vi "Process IMAQ Image (Webcam).vi"() -> ()   [LabVIEW 2020]
uses:
  <vilib>/userDefined/High Color/IMAQdx.ctl
  <vilib>/vision/driver/IMAQdx.llb/IMAQdx Buffer Number Mode.ctl
  6d5f1638-640c-4e20-b011-0cee3ae60b95.vi
  688a6956-cd2d-4b8a-a8be-e172edc5432f.vi
  45820c2d-b3f1-45d5-9983-17417cdda85c.vi
  G-Embedded-Python-Interpreter-Toolkit/Null Py Object Refnum.vi
  6d5f1638-640c-4e20-b011-0cee3ae60b95.vi/96ddca92-7bbf-40e2-a1a5-d32f291eb6af.vi
  G-Embedded-Python-Interpreter-Toolkit-IMAQ/IMAQ to Py Object.vi/22f05568-5bba-4402-9e98-aca160827363.vi
  688a6956-cd2d-4b8a-a8be-e172edc5432f.vi/6c7a13f1-33d3-431d-8188-904cac5422b3.vi
  45820c2d-b3f1-45d5-9983-17417cdda85c.vi/6c7a13f1-33d3-431d-8188-904cac5422b3.vi
  G-Embedded-Python-Interpreter-Toolkit/Python Object Reference to Pointer Sized Ref.vi
  G-Embedded-Python-Interpreter-Toolkit/Pointer Sized Ref to Python Object Reference.vi
  G-Embedded-Python-Interpreter-Toolkit/Merge Call Library Errors.vi
  G-Embedded-Python-Interpreter-Toolkit/Generate Argument Type Info.vi
  G-Embedded-Python-Interpreter-Toolkit/Create Py Object IMAQ Image.vi
  G-Embedded-Python-Interpreter-Toolkit/G-Embedded-Python-Interpreter-Toolkit.lvlib
  G-Embedded-Python-Interpreter-Toolkit-IMAQ/G-Embedded-Python-Interpreter-Toolkit-IMAQ.lvlib
  <vilib>/vision/driver/NI_Vision_Acquisition_Software.lvlib
panel:
  in  "stop":bool
  out "Image":T1(plugin-control)
  in  "Session In":T2="cam0"
  out "Print Ouptut":string
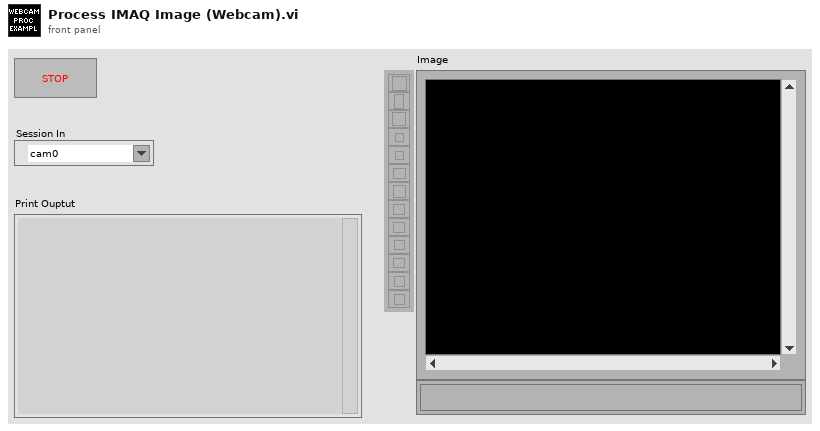
[diagram p1: front panel]
types:
  T1 = typedef "IMAQ Image.ctl" = refnum<image>
  T2 = typedef "IMAQdx.ctl" = refnum<k21>
  T3 = typedef "Image Type" = u32
  T4 = typedef "G-Embedded-Python-Interpreter-Toolkit.lvlib/Python Object Reference.ctl" = refnum<k1>
  T5 = typedef "NI_Vision_Acquisition_Software.lvlib/IMAQdx Buffer Number Mode.ctl" = enum32{"Next", "Last", "Buffer Number", "Every", "Last New"}
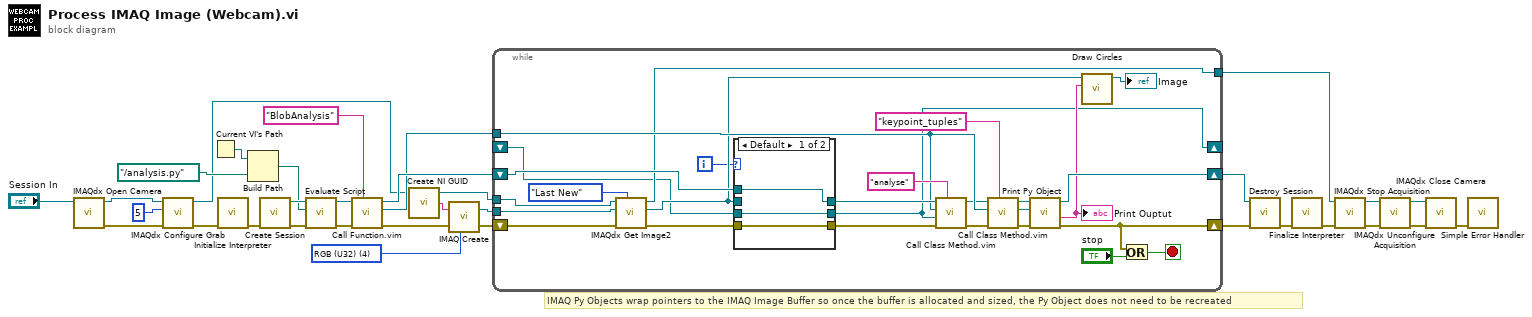
[diagram p0: block diagram]
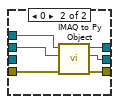
[diagram p2: hidden frame]
diagram:
  w23 = T3 4 items=["Grayscale (U8)", "Grayscale (I16)", "Grayscale (SGL)", "Complex (CSG)", "RGB (U32)", "HSL (U32)", "RGB (U64)", "Grayscale (U16)"] ("Image Type")
  # "IMAQ Py Objects wrap pointers to the IMAQ Image Buffer so once the buffer is allocated and sized, the Py Object does not need to be recreated"
  n1 = call <vilib>:"IMAQdx Open Camera.vi"("Session In"="Session In") -> ("error out"=w11:errorcluster, "Session Out"=w12:T2)  [unwired: 9 in]
  n2 = call <vilib>:"IMAQdx Configure Grab.vi"("error in"=w11, "Number of Buffers"=u32 5, "Session In"=w12) -> ("error out"=w9:errorcluster, "Session Out"=w8:T2)  [unwired: 7 in]
  n3 = Current VI's Path() -> (path=w21:path)
  n4 = call "Initialize Interpreter.vi"("error in (no error)"=w9) -> ("error out"=w32:errorcluster)  [unwired: 9 in, 1 out]
  n5 = Build Path(base path=w21, name or relative path=path "../analysis.py") -> (appended path=w28:path)
  n6 = call "Create Session.vi"("error in (no error)"=w32) -> ("error out"=w31:errorcluster, "Session Handle"=w30:refnum<data-value>)  [unwired: 9 in]
  n7 = call "Evaluate Script.vi"("error in (no error)"=w31, "Script File Path"=w28, "Session Handle in"=w30) -> ("error out"=w25:errorcluster, "Session Handle out"=w26:refnum<data-value>)  [unwired: 7 in]
  n8 = call "Call Function.vim"("Function Name"="BlobAnalysis", "error in (no error)"=w25, "Data Value Reference in"=w26) -> ("error out"=w22:errorcluster, "Returned Python Object Refnum"=w18:T4, "Data Value Reference out"=w20:refnum<data-value>)  [unwired: 6 in]
  n9 = call <vilib>:"Create NI GUID.vi"() -> ("NI GUID"=w19:string)
  n10 = call "IMAQ Create"("Image Name"=w19, "Image Type"=w23, "error in (no error)"=w22) -> ("New Image"=w14:T1, "error out"=w13:errorcluster)  [unwired: 2 in]
  n11 = while {
    tunnel: w18 -> [w54]
    tunnel: w14 -> [w47]
    shift-right: [w48] -> w17
    shift-left: w20 -> [w58]
    shift-right: [w42] -> w16
    shift-left: w13 -> [w46]
    tunnel: w8 -> [w40]
    tunnel: [w39] -> w3
    shift-right: [w34] -> _
    shift-left: _ -> [w33]
    i -> [w35]
    stop <- w43 stop-if-true
    n12 = call <vilib>:"IMAQdx Get Image2.vi"("Buffer Number Mode (Next)"=IMAQdx_Buffer_Number_Mode."Last New", "error in"=w46, "Image In"=w47, "Session In"=w40) -> ("error out"=w45:errorcluster, "Image Out"=w38:T1, "Session Out"=w39:T2)  [unwired: 4 in, 1 out]
    n13 = case shown="Default" w35 {
      tunnel: w58 -> [w60 w68]
      tunnel: [w60 w67] -> w57
      tunnel: [w62 w66] -> w56
      tunnel: [w61 w65] -> w34
      tunnel: w45 -> [w62 w64]
      tunnel: w38 -> [_ w63]
      tunnel: w33 -> [w61 _]
      frame Default {
      }
      frame 0 {
        n14 = call "IMAQ to Py Object.vi"("error in (no error)"=w64, "Image In"=w63, "Session Handle in"=w68) -> ("error out"=w66:errorcluster, "Python Object Refnum"=w65:T4, "Session Handle out"=w67:refnum<data-value>)  [unwired: 6 in]
      }
    }
    n15 = call "Call Class Method.vim"("Function Name"="analyse", "error in (no error)"=w56, "Arguments in (Default - Empty)"=w34, "Class Instance"=w54, "Data Value Reference in"=w57) -> ("error out"=w55:errorcluster, "Data Value Reference out"=w50:refnum<data-value>)  [unwired: 4 in, 1 out]
    n16 = call "Call Class Method.vim"("Function Name"="keypoint_tuples", "error in (no error)"=w55, "Class Instance"=w54, "Data Value Reference in"=w50) -> ("error out"=w53:errorcluster, "Returned Python Object Refnum"=w51:T4, "Data Value Reference out"=w49:refnum<data-value>)  [unwired: 5 in]
    n17 = call "Print Py Object.vi"("error in (no error)"=w53, "Python Object Refnum in"=w51, "Session Handle in"=w49) -> ("error out"=w42:errorcluster, "Print Ouptut"=w36:string, "Session Handle out"=w48:refnum<data-value>)  [unwired: 5 in, 1 out]
    "Print Ouptut" <- w36
    n18 = call "Draw Circles.vi"("Print Ouptut"=w36, "Refnum in"=w38) -> ("Refnum out"=→"Image":T1)  [unwired: 9 in]
    n19 = Or(x=w42, y="stop") -> (x .or. y?=w43:bool)
  }
  n20 = call "Destroy Session.vi"("error in (no error)"=w16, "Session Handle"=w17) -> ("error out"=w24:errorcluster)  [unwired: 9 in]
  n21 = call "Finalize Interpreter.vi"("error in (no error)"=w24) -> ("error out"=w2:errorcluster)  [unwired: 10 in]
  n22 = call <vilib>:"IMAQdx Stop Acquisition.vi"("error in"=w2, "Session In"=w3) -> ("error out"=w7:errorcluster, "Session Out"=w6:T2)  [unwired: 8 out]
  n23 = call <vilib>:"IMAQdx Unconfigure Acquisition.vi"("error in"=w7, "Session In"=w6) -> ("error out"=w4:errorcluster, "Session Out"=w5:T2)  [unwired: 8 out]
  n24 = call <vilib>:"IMAQdx Close Camera.vi"("error in"=w4, "Session In"=w5) -> ("error out"=w1:errorcluster)  [unwired: 9 out]
  n25 = call <vilib>:"Simple Error Handler.vi"("error in (no error)"=w1) -> ()  [unwired: 4 in, 5 out]
